vi "Initialize.vi"(8 "error in":errorcluster, 10 "parameters":variant, 11 "node in":refnum<class "control module editor.lvclass">) -> (0 "error out":errorcluster, 2 "summary":T2[](array[typedef]), 3 "data value reference":T1)   [LabVIEW 2013, in "control module editor.lvclass"]
doc: "Initializes the data of a node to its default state.\nThe object is not created inside of this VI, because it is created from a File depending on user selection."
uses:
  control module editor.lvclass
  <vilib>/NI/Configuration Framework/Node/Summary.ctl
  <vilib>/NI/Configuration Framework/Node/NodeRef.ctl
  <vilib>/NI/Configuration Framework/Node/NISE_CEF_Node.lvclass
  Configuration Editor/Classes/Module editor node/module editor node.lvclass
  configuration/control module configuration.lvclass
  configuration/control module configuration.lvclass/control module configuration.ctl
  read fixed channel configuration.vi
  <vilib>/NI/Configuration Framework/NISE_CEF_TreeControl.lvlib
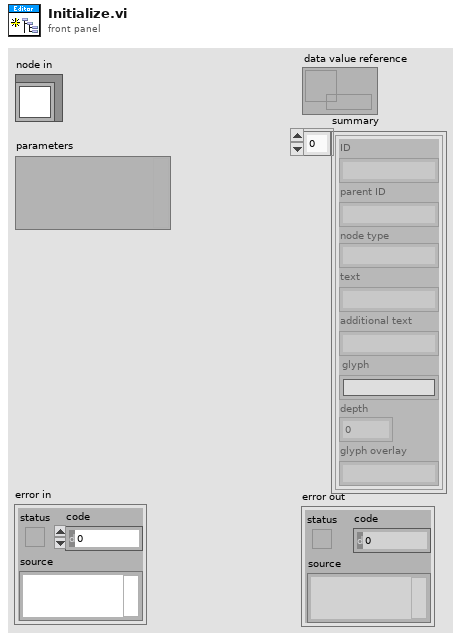
[diagram p1: front panel]
types:
  T1 = typedef "NISE_CEF_Node.lvclass/NodeRef.ctl" = refnum<data-value>
  T2 = typedef "NISE_CEF_Node.lvclass/Summary.ctl" = cluster{"ID":string, "parent ID":string, "node type":string, "text":string, "additional text":string, "glyph":string, "depth":i32, "glyph overlay":string}
  T3 = typedef "control module configuration.lvclass/error classification setting.ctl" = cluster{"code":i32, "error classification":T4}
  T4 = typedef "TBM module execution interface.lvclass/error classification.ctl" = enum16{"unknown", "none", "trivial", "recoverable", "critical"}
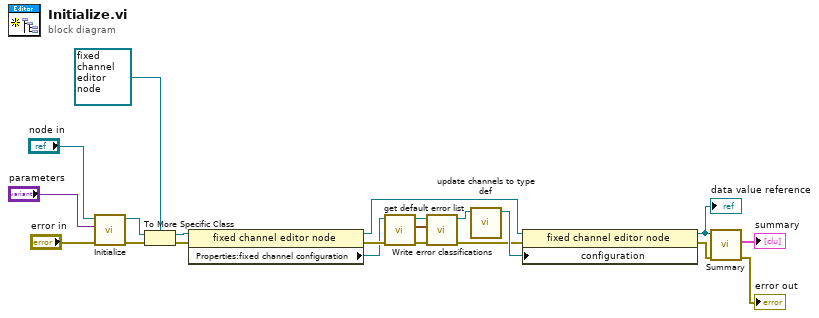
[diagram p0: block diagram]
diagram:
  n1 = call-parent "Initialize.vi"("error in"="error in", "parameters"="parameters", "node in"="node in") -> ("error out"=w21:errorcluster, "data value reference"=w17:T1)  [unwired: 6 in, 1 out]
  n2 = To More Specific Class(target class=refnum<data-value> refnum, reference=w17, error in=w21) -> (specific class reference=w12:refnum<data-value>, error out=w15:errorcluster)
  n3 = property class="fixed channel editor node"(reference=w12, error in=w15) -> (reference out=w10:refnum<data-value>, error out=w4:errorcluster, "Properties:fixed channel configuration"=w3:refnum<class "control module configuration.lvclass">)
  n4 = call-dynamic "get default error list.vi"("error in (no error)"=w4, "fixed channel configuration in"=w3) -> ("error out"=w5:errorcluster, "error list"=w6:T3[], "fixed channel configuration out"=w7:refnum<class "control module configuration.lvclass">)  [unwired: 7 in]
  n5 = call "Write error classifications.vi"("error in"=w5, "error classifications"=w6, "control module configuration in"=w7) -> ("error out"=w1:errorcluster, "control module configuration out"=w2:refnum<class "control module configuration.lvclass">)  [unwired: 7 in]
  n6 = call-dynamic "update channels to type def.vi"("fixed channel configuration in"=w2) -> ("fixed channel configuration out"=w8:refnum<class "control module configuration.lvclass">)  [unwired: 10 in]
  n7 = property class="fixed channel editor node"(reference=w10, error in=w1, "configuration"=w8) -> (reference out=w9:refnum<data-value>, error out=w11:errorcluster)
  "data value reference" <- w9
  n8 = call <vilib>:"Summary.vi"("error in"=w11, "node self ref"=w9) -> ("error out"=→"error out":errorcluster, "summary"=→"summary":T2[])  [unwired: 8 in]
